vi "Signals.Scale.Raw.vi"(5 "Lookup":variant, 6 "Type":T1, 7 "Writes Ref":T2, 8 "error in":errorcluster, 11 "ID":u32) -> (0 "error out":errorcluster, 2 "Data":u8[](array[numeric]))   [LabVIEW 2024, in "Diagnostics Addon Engine.lvlib"]
uses:
  Diagnostics Addon Engine.lvlib
  <vilib>/NI/NIVS Inline Async API/_Data Access Engine/Data Access Engine/Types/Read.DVR.ctl
  <vilib>/NI/NIVS Inline Async API/_Data Access Engine/Access Type Classes/Read/Read.lvclass
  Addon Shared/Types/Type.ctl
  Addon Shared/Types/Frame.Lookup.Info.ctl
  <vilib>/NI/NIVS Inline Async API/_Data Access Engine/Access Type Classes/Read/Read.lvclass/Read.ctl
  <vilib>/NI/NIVS Inline Async API/_Data Access Engine/Data Access Engine/Methods/Read.Data.vi
  <vilib>/NI/NIVS Inline Async API/_Data Access Engine/Access Type Classes/Read/Read.ProcessData.vi
  Addon Shared/SubVIs/Constants.vi
  <vilib>/xnet/xnet.llb/XNET Convert (Signal to Frame CAN).vi
  Addon Shared/Diagnostics Addon Shared.lvlib
  <vilib>/NI/NIVS Inline Async API/_Data Access Engine/Data Access Engine/Data Access Engine.lvclass
  <vilib>/Utility/SystemLogging/NI_SystemLogging.lvlib
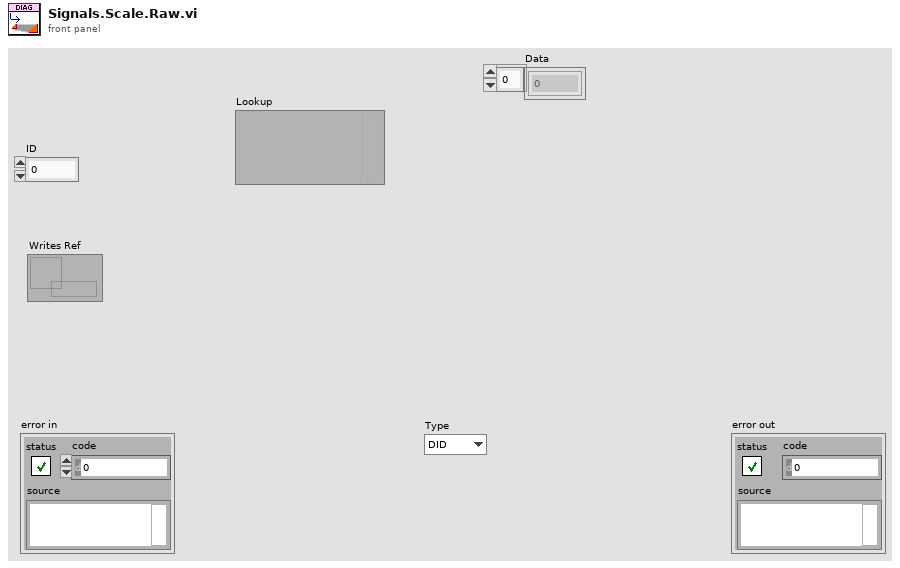
[diagram p1: front panel]
types:
  T1 = typedef "Diagnostics Addon Shared.lvlib/Type.ctl" = enum16{"DID", "CDID", "PID", "CPID", "Read Memory", "Write Memory", "IO Control", "Routine Start", "Routine Request", "Routine Stop", "User Defined", "DTC Control", "Clear DTCs", "Read DTCs", "Start DTCs", "DTC Change Count", "Tester Present", "Unlock ECU", "Reset ECU", "Diag Session Control", "Communication Control", "DPID Control", "Poll Control", "Diag Comm Port Control"}
  T2 = typedef "Data Access Engine.lvlib/Data Access Engine.lvclass/Read.DVR.ctl" = refnum<data-value>
  T3 = enum16{"Output/Write", "Input/Read", "Input/ReadWrite"}
  T4 = typedef "Diagnostics Addon Shared.lvlib/Frame.Lookup.Info.ctl" = cluster{"Offset":i32, "Length":i32, "ByteLength":u16}
  T5 = typedef "XNET Frame CAN.ctl" = cluster{"timestamp":timestamp, "payload":u8[], "identifier":u32, "type":T6, "extended?":bool, "echo?":bool}
  T6 = typedef "XNET Frame Type CAN.ctl" = u8
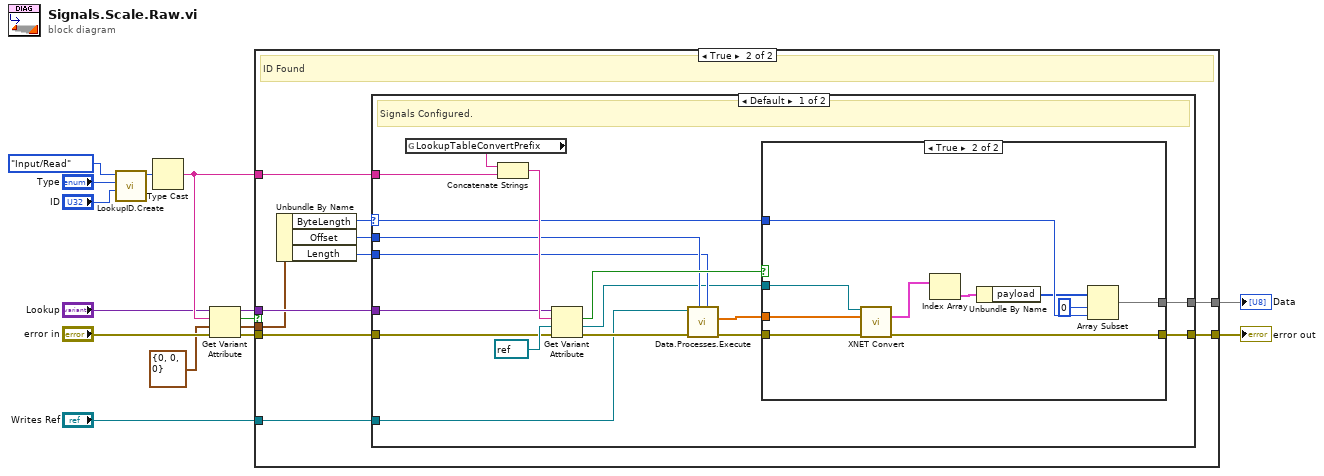
[diagram p0: block diagram]
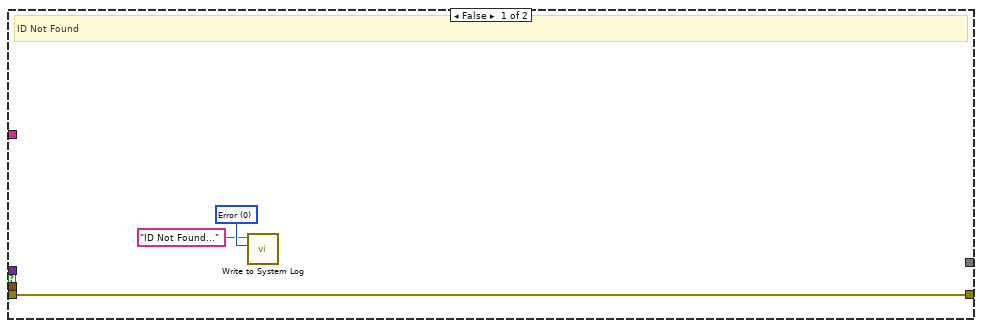
[diagram p2: hidden frame]
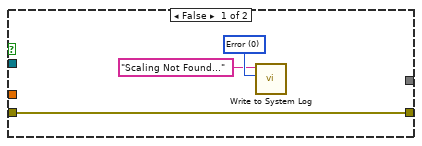
[diagram p3: hidden frame]
diagram:
  n1 = call "LookupID.Create.vi"("Serivce ID"="ID", "Service Type"="Type", "Direction"=T3."Input/Read") -> ("Result"=w5:u64)  [unwired: 8 in]
  n2 = Type Cast(x=w5) -> (*(type *) &x=w12:string)  [unwired: 1 in]
  n3 = Get Variant Attribute(Variant="Lookup", name=w12, default value (empty Variant)=T4 {"Offset"=0, "Length"=0, "ByteLength"=0} ("cluster"), error in="error in") -> (duplicate Variant=w11:variant, found=w1:bool, value=w2:T4, error out=w13:errorcluster)
  n4 = case shown="True" w1 {
    tunnel: w13 -> [w18 w28]
    tunnel: w12 -> [_ w27]
    tunnel: w11 -> [_ w26]
    tunnel: [w18 w25] -> w9
    tunnel: "Writes Ref" -> [_ w22]
    tunnel: [_ w21] -> w3
    tunnel: w2 -> [_ w20]
    frame False {
      w17 = 0 items=["Error", "Warning", "Informational"] ("severity")
      # "ID Not Found"
      n5 = call <vilib>:"Write to System Log.vi"("severity"=w17, "message"="ID Not Found..." ("Message")) -> ()  [unwired: 9 in, 1 out]
    }
    frame True {
      # "ID Found"
      n6 = Unbundle By Name(w20) -> ("ByteLength"=w19:u16, "Offset"=w24:i32, "Length"=w23:i32)
      n7 = case shown="Default" w19 {
        selector: w19 -> [w29 _]
        tunnel: w28 -> [w42 w59]
        tunnel: w27 -> [w41 _]
        tunnel: w26 -> [w40 _]
        tunnel: [w39 w59] -> w25
        tunnel: w24 -> [w37 _]
        tunnel: w23 -> [w36 _]
        tunnel: w22 -> [w33 _]
        tunnel: [w31 _] -> w21
        frame Default {
          # "Signals Configured."
          n8 = global read "Constants.vi" "LookupTableConvertPrefix"() -> (w43:string)
          n9 = Concatenate Strings(w43, w41) -> (w44:string)
          n10 = Get Variant Attribute(Variant=w40, name=w44, default value (empty Variant)=refnum<k21> refnum ("DID Conversion"), error in=w42) -> (found=w38:bool, value=w30:refnum<k21>, error out=w35:errorcluster)  [unwired: 1 out]
          n11 = call-poly <vilib>:"Data.Processes.Execute.vi"("length"=w36, "index"=w37, "error in (no error)"=w35, "Ref"=w33) -> ("error out"=w34:errorcluster, "Values"=w32:dbl[])  [unwired: 5 in, 1 out]
          n12 = case shown="True" w38 {
            tunnel: w34 -> [w48 w58]
            tunnel: [w48 w52] -> w39
            tunnel: w32 -> [_ w54]
            tunnel: w30 -> [_ w57]
            tunnel: w29 -> [_ w55]
            tunnel: [_ w53] -> w31
            frame False {
              w47 = 0 items=["Error", "Warning", "Informational"] ("severity")
              n13 = call <vilib>:"Write to System Log.vi"("severity"=w47, "message"="Scaling Not Found..." ("Message")) -> ()  [unwired: 9 in, 1 out]
            }
            frame True {
              n14 = call-poly <vilib>:"XNET Convert.vi"("session in"=w57, "signal data"=w54, "error in (no error)"=w58) -> ("frame data"=w51:T5[], "error out"=w52:errorcluster)  [unwired: 9 in, 2 out]
              n15 = Index Array(array=w51) -> (element=w50:T5)  [unwired: 1 in]
              n16 = Unbundle By Name(w50) -> ("payload"=w49:u8[])
              n17 = Array Subset(array=w49, index=0, length=w55) -> (w53:u8[])
            }
          }
        }
        frame 0 {
          # "No Signals Configured."
        }
      }
    }
  }
  "error out" <- w9
  "Data" <- w3
